vi "Frequency Response - Digital Mic.vi"() -> ()   [LabVIEW 2022 SP3]
uses:
  <vilib>/PDM Acquisition Toolkit/host/Classes/Session/Controls/Logic Levels.ctl
  <vilib>/PDM Acquisition Toolkit/shared/controls/decimation order.ctl
  <vilib>/PDM Acquisition Toolkit/host/Classes/Tasks/PDM Tasks/Controls/Acquisition Mode.ctl
  <vilib>/PDM Acquisition Toolkit/shared/controls/clock mode.ctl
  <vilib>/PDM Acquisition Toolkit/host/API/Controls/PDM Digital Start Trigger Cluster.ctl
  <vilib>/PDM Acquisition Toolkit/shared/controls/PXI trigger lines.ctl
  <vilib>/PDM Acquisition Toolkit/shared/controls/trigger polarity.ctl
  source/shared/measurements/controls/units settings - mic.ctl
  source/shared/measurements/controls/measurement units.ctl
  source/shared/measurements/controls/single tone microphone measurement settings.ctl
  <vilib>/addons/_NISVFA/_Generation/Signal Generation/SV Signal/SV Signal.lvclass/SV Signal.ctl
  <vilib>/DAQmx/write.llb/DAQmx Write (Analog Wfm 1Chan NSamp).vi
  <vilib>/DAQmx/read.llb/DAQmx Read (Analog 1D Wfm NChan NSamp).vi
  <vilib>/addons/_NISVFA/_Generation/Signal Generation/SV Signal/Write Leading Synchronization Pulse Enable.vi
  <vilib>/addons/_NISVFA/_Generation/Signal Generation/SV Signal/Write Synchronization Pulse Duration.vi
  <vilib>/addons/_NISVFA/_Generation/Signal Generation/SV Signal/Read Total Samples.vi
  Program Files/NI/LVAddons/nisvt/1/examples/Sound and Vibration/Audio Measurements/subVIs/sv_Align Waveforms by Leading Sync Pulse.vi
  <vilib>/addons/_NISVFA/_Generation/Signal Generation/SV Signal/Read Synchronization Pulse Waveform.vi
  <vilib>/addons/_NISVFA/_Shared subVIs/Common/svc_Check for Waveform Parameter Continuity (N Ch).vi
  Program Files/NI/LVAddons/nisvt/1/examples/Sound and Vibration/Audio Measurements/subVIs/sv_Append Virtual Reference.vi
  <vilib>/addons/_NISVFA/_Generation/Signal Generation/SV Signal/Calculate Number of Remaining Samples.vi
  Program Files/NI/LVAddons/nisvt/1/examples/Sound and Vibration/Audio Measurements/subVIs/sv_Measure Delay for Active and Idle Channels.vi
  <vilib>/addons/_NISVFA/_Generation/Signal Generation/SV Signal/Read Leading Synchronization Pulse Enable.vi
  <vilib>/addons/_NISVFA/_Generation/Signal Generation/SV Signal/Read Trailing Synchronization Pulse Enable.vi
  <vilib>/addons/_NISVFA/_Shared subVIs/Common/svc_Check for Waveform Parameter Continuity (no state).vi
  <vilib>/addons/_NISVFA/_Shared subVIs/Common/sv_Get NI Property Name String.vi
  <vilib>/addons/Sound and Vibration/svt_Calibration/SV Measure Delay and Polarity and Coherence (Nx1).vi
  Program Files/NI/LVAddons/nisvt/1/examples/Sound and Vibration/Audio Measurements/subVIs/sv_Assign Delay to Idle Channels.vi
  <vilib>/addons/_NISVFA/_Shared subVIs/Common/svc_Get SV Channel Info.vi
  <vilib>/addons/Sound and Vibration/svt_Calibration/SV Measure Delay and Polarity and Coherence.vi
  <vilib>/addons/_NISVFA/_Shared subVIs/Common/svc_Unit Label to Engineering Units.vi
  <vilib>/addons/_NISVFA/_Shared subVIs/Common/svc_Engineering Units to Unit Label.vi
  <vilib>/Analysis/_algsub.llb/Vector Norm.vi
  <vilib>/Analysis/_algsub.llb/Real Vector Norm.vi
  <vilib>/addons/_NISVFA/_Shared subVIs/Common/SV Get Data Subset.vi
  <vilib>/addons/_NISVFA/_Shared subVIs/Common/svc_Get Array Subset (Index).vi
  <vilib>/addons/_NISVFA/_Shared subVIs/Common/svc_Coerce Index and Length.vi
  <vilib>/addons/_NISVFA/_Shared subVIs/Common/svc_Conditional Merge Error.vi
  <vilib>/addons/_NISVFA/_Generation/Signal Generation/SV Discrete Sweep/SV Discrete Sweep.lvclass
  C:/Program Files/NI/LVAddons/nisvt/1/vi.lib/addons/_NISVFA/_Generation/Signal Generation/SV Signal/SV Signal.lvclass
  C:/Program Files/NI/LVAddons/nisvt/1/vi.lib/addons/_NISVFA/_Generation/Signal Generation/SV Function/SV Function.lvclass
  <vilib>/addons/_NISVFA/_Generation/Signal Generation/SV Discrete Sweep/Configure Frequency Sweep at Constant Amplitude.vi
  <vilib>/PDM Acquisition Toolkit/host/API/Public/Create Tasks/Create PDM Input Task.vi
  <vilib>/addons/_NISVFA/_Generation/Signal Generation/SV Signal/Write Ramp Parameters.vi
  <vilib>/addons/_NISVFA/_Generation/Signal Generation/SV Signal/Write Measurement Duration.vi
  <vilib>/addons/_NISVFA/_Generation/Signal Generation/SV Function/Write Measurement Cycles.vi
  <vilib>/addons/_NISVFA/_Generation/Signal Generation/SV Signal/Write Pre-Measurement Settling Duration.vi
  <vilib>/addons/_NISVFA/_Generation/Signal Generation/SV Function/Write Pre-Measurement Settling Cycles.vi
  <vilib>/addons/_NISVFA/_Generation/Signal Generation/SV Signal/Read Sample Rate.vi
  <vilib>/addons/_NISVFA/_Generation/Signal Generation/SV Signal/Read Generation State.vi
  <vilib>/addons/_NISVFA/_Generation/Signal Generation/SV Signal/Read System Timing Model.vi
  <vilib>/PDM Acquisition Toolkit/host/API/Public/Configure/Timing/Configure Timing - PDM Input.vi
  <vilib>/PDM Acquisition Toolkit/host/API/Public/Configure/PDM Channel/Configure Microphone Sensitivity DBFS.vi
  <vilib>/PDM Acquisition Toolkit/host/API/Public/Configure/Triggering/Configure PDM Trigger (Digital Edge).vi
  <vilib>/DAQmx/create/channels.llb/DAQmx Create Channel (AO-Voltage-Basic).vi
  <vilib>/DAQmx/configure/timing.llb/DAQmx Timing (Sample Clock).vi
  <vilib>/DAQmx/configure/events/hardwareSignals.llb/DAQmx Export Signal (Most Signals).vi
  <vilib>/DAQmx/create/channels.llb/DAQmx Create Channel (AI-Sound Pressure-Microphone).vi
  <vilib>/DAQmx/configure/trigger.llb/DAQmx Start Trigger (Digital Edge).vi
  <vilib>/DAQmx/miscellaneous.llb/DAQmx Fill In Error Info.vi
  <vilib>/PDM Acquisition Toolkit/host/API/Public/Read/Read PCM Waveform.vi
  <vilib>/PDM Acquisition Toolkit/host/API/Public/Clear/Clear PDM Input Task.vi
  <vilib>/addons/_NISVFA/_Generation/Signal Generation/SV Signal/Write System Timing Model.vi
  <vilib>/addons/_NISVFA/_Shared subVIs/Data Objects/Waveforms (DBL)/SV Read Newest Data.vi
  <vilib>/measure/maresamp.llb/Resample Waveforms (single shot).vi
  <vilib>/measure/maresamp.llb/Resample Waveform (single shot).vi
  <vilib>/addons/_NISVFA/_Shared subVIs/Common/svc_Check dt for Equal Sample Rates.vi
  <vilib>/Waveform/TSOps.llb/Timestamp Subtract.vi
  <vilib>/Analysis/2dsp.llb/CrossCorrelation.vi
  <vilib>/Analysis/2dsp.llb/1D Cross Correlation (DBL).vi
  <vilib>/addons/_NISVFA/_Shared subVIs/Common/svc_Fit Quadratic to Max Three Points in Array.vi
  <vilib>/Utility/error.llb/Error Cluster From Error Code.vi
  <vilib>/addons/_NISVFA/_Shared subVIs/Common/svc_Caller VI Returned in Error Source.vi
  <vilib>/addons/_NISVFA/_Shared subVIs/Common/SV Remove Delays (1,N) from Waveforms (N Ch) (DBL).vi
  <vilib>/addons/_NISVFA/_Shared subVIs/Common/SV Remove Delays from Waveforms.vi
  <vilib>/addons/_NISVFA/_Shared subVIs/Data Objects/Waveforms (DBL)/SV Read Next Measurement Data.vi
  <vilib>/addons/_NISVFA/_Generation/Signal Generation/SV Signal/SV Signal.lvclass
  <resource>/objmgr/daqmx.rc
  <vilib>/addons/_NISVFA/_Shared subVIs/Data Objects/Waveforms (DBL)/Waveforms (N Ch).lvclass
  Program Files/NI/LVAddons/nisvt/1/examples/Sound and Vibration/SoundVib_Audio Examples.lvlib
  C:/Program Files/NI/LVAddons/nisvt/1/vi.lib/addons/_NISVFA/_Generation/Signal Generation/SV Sinusoid/SV Sinusoid.lvclass
  C:/Program Files/NI/LVAddons/nisvt/1/vi.lib/addons/_NISVFA/_Generation/Signal Generation/SV Discrete Sweep/SV Discrete Sweep.lvclass
  <vilib>/PDM Acquisition Toolkit/host/API/PDM Acquisition Toolkit.lvlib
  <vilib>/PDM Acquisition Toolkit/host/Classes/Tasks/PDM Tasks/PDM Task.lvclass
  <vilib>/PDM Acquisition Toolkit/shared/PDM Shared.lvlib
  <vilib>/PDM Acquisition Toolkit/host/Classes/Session/DecoderSession.lvclass
panel:
  out "duration (s)":dbl
  out "Sample Rate (Hz)":dbl
  in  "Tab Control":T1(tab)=enum."Frequency Response"
  out "Waveform Graph":waveform(dbl)[](graph)=[{"t0"=timestamp(3812131384.799704 s since 1904-01-01), "dt"=1.9531249997269942e-05, "Y"=array[65939 elements], "attributes"=variant("NI_ChannelName"=variant(string "PXI1Slot2/ai0"), "NI_UnitDescription"=variant(string "Pascals"), "NI_dBReference"=variant(dbl 2e-05))}]
  out "XY Graph":cluster{"X":dbl[], "Y":dbl[]}[](graph)
  out "Distortion":cluster{"X":dbl[], "Y":dbl[]}[](graph)
  in  "sweep settings":T2(tab)=enum."Source Settings"
  in  "PDM Channels":string="PXI1Slot5\\PDMi 0"
  in  "Logic Level":T3
  in  "Decimation Factor":T4=64 items=["24"=24, "32"=32, "48"=48, "64"=64, "96"=96, "128"=128]
  in  "PDM Clock Rate":dbl=3072000.0 format="%#_6p"
  in  "Microphone Sensitivity (dBFS)":dbl=-26.0 format="%#_13g"
  out "Actual PDM Clock Rate":dbl=3071999.9922439456 format="%#_6p"
  out "Actual PCM Clock Rate":dbl=47999.99987881165 format="%#_6p"
  in  "physical channels":tag
  in  "microphone sensitivity":dbl=10.0
  in  "number of steps":i32=50 min=1
  in  "amplitude":dbl=94.0 format="%.2p dBSPL"
  in  "frequency spacing":enum16{"Linear", "Logarithmic"}(ring)=enum."Logarithmic"
  in  "sweep range":cluster{"start":dbl, "stop":dbl}={"start"=10000.0, "stop"=300.0} {"stop" min=0.0 format="%.2f"; "start" min=0.0 format="%.2f"}
  in  "output voltage ratio":dbl=0.914 format="%#_g Pa/V"
  in  "speaker excitation channel":tag="PXI1Slot2/ao0"
  in  "measurement":cluster{"time":dbl, "cycles":dbl}={"time"=0.001, "cycles"=25.0} {"cycles" min=5.0 max=1000.0 step=1.0; "time" min=0.0 max=5.0 step=0.0001 format="%.3f s"}
  in  "settling":cluster{"time":dbl, "cycles":dbl}={"time"=0.0, "cycles"=1.0} {"cycles" min=0.0 max=100.0 step=0.5; "time" min=0.0 max=5.0 step=0.0001 format="%.3f s"}
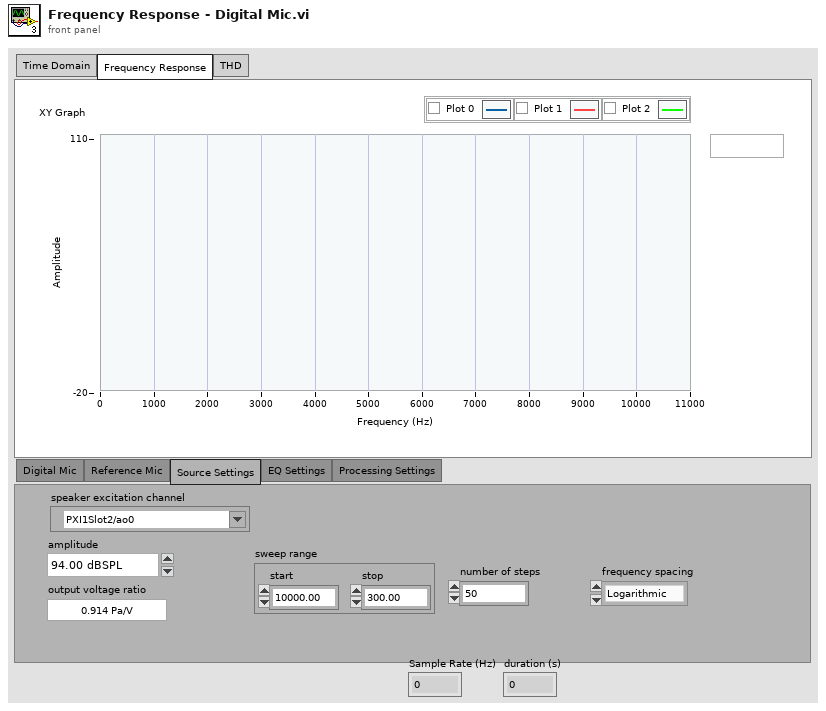
[diagram p1: front panel]
types:
  T1 = enum32{"Time Domain", "Frequency Response", "THD"}
  T2 = enum32{"Digital Mic", "Reference Mic", "Source Settings", "EQ Settings", "Processing Settings"}
  T3 = typedef "PDM Acquisition Class Library.lvlib/DecoderSession.lvclass/Logic Levels.ctl" = enum16{"3.3 V", "1.8 V", "1.2 V"}
  T4 = typedef "PDM Shared.lvlib/decimation order.ctl" = u16
  T5 = typedef "PDM Acquisition Toolkit.lvlib/PDM Digital Start Trigger Cluster.ctl" = cluster{"source":T6, "polarity":T7}
  T6 = typedef "PDM Shared.lvlib/PXI trigger lines.ctl" = enum16{"PXI_Trig0", "PXI_Trig1", "PXI_Trig2", "PXI_Trig3", "PXI_Trig4", "PXI_Trig5", "PXI_Trig6", "PXI_Trig7"}
  T7 = typedef "PDM Shared.lvlib/trigger polarity.ctl" = enum16{"Rising Edge", "Falling Edge"}
  T8 = typedef "PDM Shared.lvlib/clock mode.ctl" = enum16{"divided clock", "DDS"}
  T9 = typedef "PDM Acquisition Class Library.lvlib/PDM Task.lvclass/Acquisition Mode.ctl" = enum16{"Finite", "Continuous"}
  T10 = cluster{"profile":enum16{"Linear", "Half cosine"}, "durations [s]":cluster{"ramp-up":dbl, "transition":dbl, "ramp-down":dbl}}
  T11 = typedef "single tone microphone measurement settings.ctl" = cluster{"Band start":dbl, "Band stop":dbl, "Frequency":dbl}
  T12 = typedef "units settings - mic.ctl" = cluster{"SNR units":T13, "THD+N units":T13, "THD units":T13}
  T13 = typedef "measurement units.ctl" = enum32{"dB", "%", "x/y"}
  T14 = typedef "single tone microphone measurements.ctl" = cluster{"channel":string, "frequency (Hz)":dbl, "amplitude (Pa rms)":dbl, "amplitude (dBSPL)":dbl, "SNR":dbl, "THD+N":dbl, "THD":dbl, "phase (deg)":dbl}
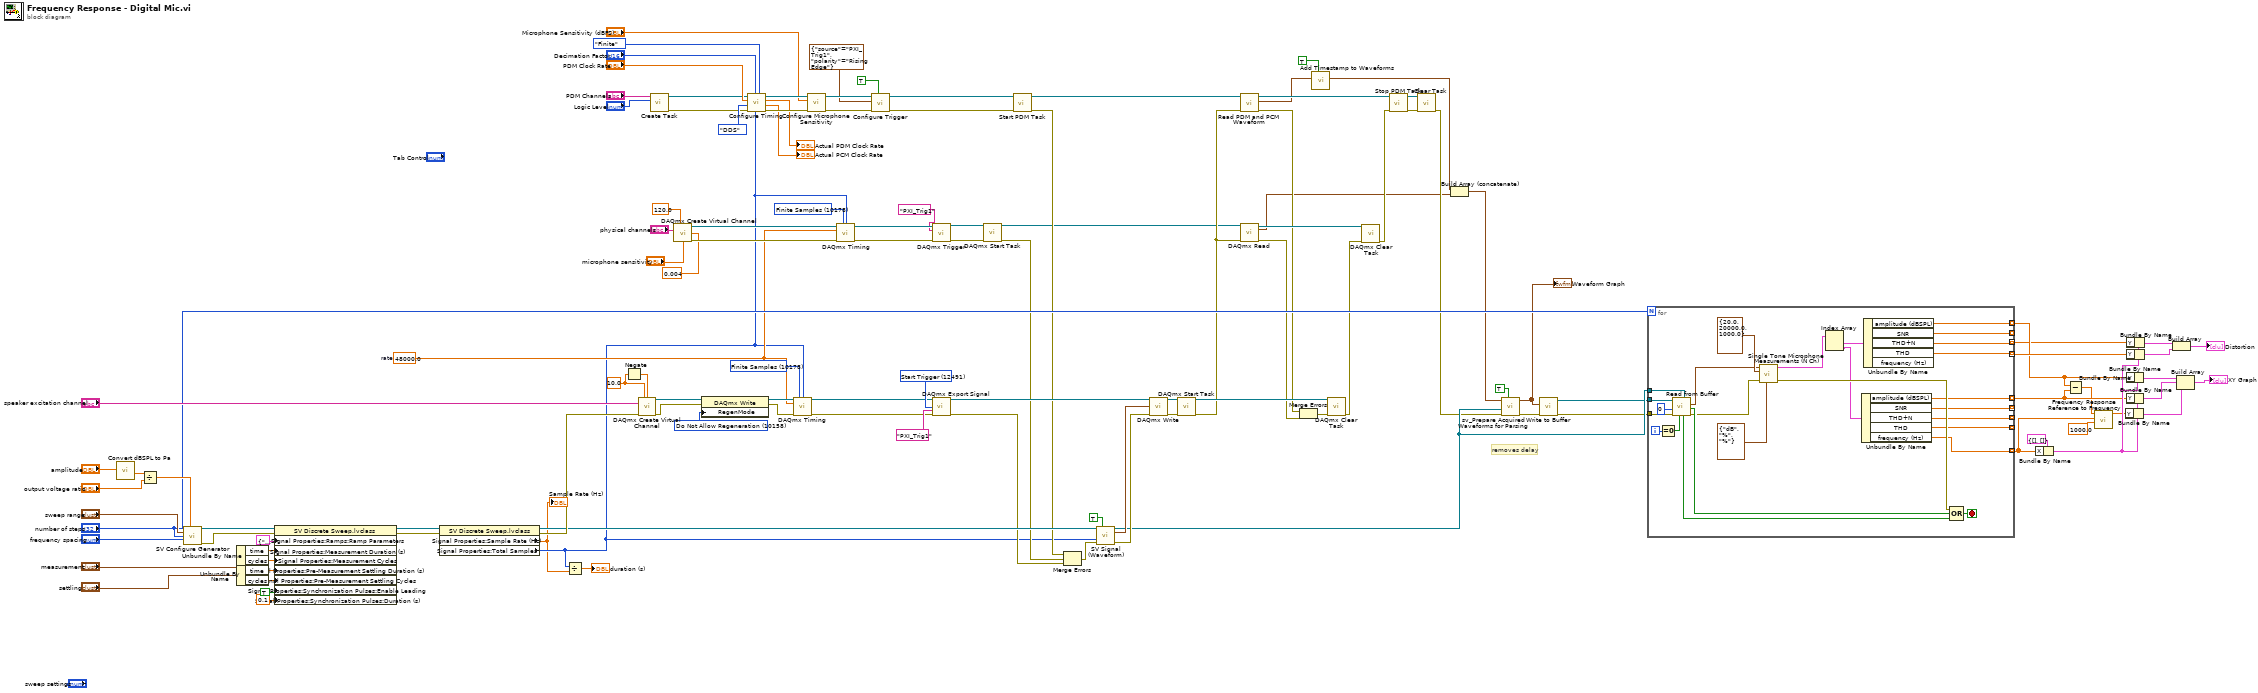
[diagram p0: block diagram]
diagram:
  w44 = 10178 items=["Finite Samples"=10178, "Continuous Samples"=10123, "Hardware Timed Single Point"=12522] ("sample mode")
  w80 = 12491 items=["AI Convert Clock"=12484, "10MHz Reference Clock"=12536, "20MHz Timebase Clock"=12486, "Sample Clock"=12487, "Advance Trigger"=12488, "Reference Trigger"=12490, "Start Trigger"=12491, "Advance Complete Event"=12492, "AI Hold Complete Event"=12493, "Counter Output Event"=12494, "Change Detection Event"=12511, "Watchdog Timer Expired Event"=12512] ("signal")
  w105 = 10158 items=["Allow Regeneration"=10097, "Do Not Allow Regeneration"=10158] ("RegenMode")
  w107 = 10.0 ("maximum value")
  w108 = 10178 items=["Finite Samples"=10178, "Continuous Samples"=10123, "Hardware Timed Single Point"=12522] ("sample mode")
  w39 = 48000.0  # rate
  # "removes delay"
  n1 = call "Convert dBSPL to Pa.vi"("dB SPL"="amplitude") -> ("Pa pk"=w81:dbl)  [unwired: 9 in, 1 out]
  n2 = Divide(x=w81, y="output voltage ratio") -> (x/y=w109:dbl)
  n3 = call-poly <vilib>:"SV Configure Generator.vi"("amplitude"=w109, "frequency range [Hz]"="sweep range", "number of steps"="number of steps", "profile"="frequency spacing") -> ("signal configuration"=w117:refnum<class "SV Discrete Sweep.lvclass">, "error out"=w116:errorcluster)  [unwired: 10 in]
  n4 = Unbundle By Name("measurement") -> ("time"=w119:dbl, "cycles"=w118:dbl)
  n5 = Unbundle By Name("settling") -> ("time"=w121:dbl, "cycles"=w120:dbl)
  n6 = property class="SV Discrete Sweep.lvclass"(reference=w117, error in=w116, "Signal Properties:Ramps:Ramp Parameters"=T10 {"profile"=enum."Half cosine", "durations [s]"={"ramp-up"=0.01, "transition"=0.0, "ramp-down"=0.01}} ("Ramp Parameters"), "Signal Properties:Measurement Duration (s)"=w119, "Signal Properties:Measurement Cycles"=w118, "Signal Properties:Pre-Measurement Settling Duration (s)"=w121, "Signal Properties:Pre-Measurement Settling Cycles"=w120, "Signal Properties:Synchronization Pulses:Enable Leading"=TRUE ("Synchronization Pulses:Enable Leading"), "Signal Properties:Synchronization Pulses:Duration (s)"=0.1 ("Synchronization Pulses:Duration")) -> (reference out=w97:refnum<class "SV Discrete Sweep.lvclass">, error out=w98:errorcluster)
  n7 = property on="Property Node" class="SV Discrete Sweep.lvclass"(reference=w97, error in=w98) -> (reference out=w94:refnum<class "SV Discrete Sweep.lvclass">, error out=w96:errorcluster, "Signal Properties:Sample Rate (Hz)"=w2:dbl, "Signal Properties:Total Samples"=w3:i32)
  "Sample Rate (Hz)" <- w2
  n8 = Divide(x=w3, y=w2) -> (x/y=→"duration (s)":dbl)
  n9 = Negate(x=w107) -> (-x=w106:dbl)
  n10 = call-poly <vilib>:"DAQmx Create Virtual Channel.vi"("maximum value"=w107, "minimum value"=w106, "physical channels"="speaker excitation channel", "error in"=w96) -> ("task out"=w104:refnum<k21>, "error out"=w102:errorcluster)  [unwired: 10 in]
  n11 = call-poly <vilib>:"Create Task.vi"("logic level"="Logic Level", "channel list"="PDM Channels") -> ("error out"=w64:errorcluster, "PDM input task out"=w65:refnum<data-value>)  [unwired: 8 in]
  n12 = call-poly <vilib>:"DAQmx Create Virtual Channel.vi"("maximum sound pressure level"=120.0, "physical channels"="physical channels", "current excitation value"=0.004, "microphone sensitivity"="microphone sensitivity") -> ("task out"=w46:refnum<k21>, "error out"=w45:errorcluster)  [unwired: 10 in]
  n13 = property class="DAQmx Write"(reference=w104, error in=w102, "RegenMode"=w105) -> (reference out=w103:refnum<k21>, error out=w101:errorcluster)
  n14 = call-poly <vilib>:"Configure Timing.vi"("acquisition mode"=Acquisition_Mode."Finite" ("Acquisition Mode"), "number of PCM samples"=w3, "decimation factor"="Decimation Factor", "error in"=w64, "clock mode"=clock_mode."DDS" ("Clock Type"), "PDM clock rate"="PDM Clock Rate", "PDM input task in"=w65) -> ("error out"=w67:errorcluster, "actual PCM clock rate"=→"Actual PCM Clock Rate":dbl, "actual PDM clock rate"=→"Actual PDM Clock Rate":dbl, "PDM input task out"=w68:refnum<data-value>)  [unwired: 1 in]
  n15 = call-poly <vilib>:"DAQmx Timing.vi"("task/channels in"=w103, "sample mode"=w108, "samples per channel"=w3, "rate"=w39, "error in"=w101) -> ("task out"=w76:refnum<k21>, "error out"=w75:errorcluster)  [unwired: 9 in]
  n16 = call-poly <vilib>:"Configure Microphone Sensitivity.vi"("error in"=w67, "microphone sensitivity (dBFS)"="Microphone Sensitivity (dBFS)", "PDM input task in"=w68) -> ("error out"=w58:errorcluster, "PDM input task out"=w61:refnum<data-value>)  [unwired: 7 in]
  n17 = call-poly <vilib>:"DAQmx Timing.vi"("task/channels in"=w46, "sample mode"=w44, "samples per channel"=w3, "rate"=w39, "error in"=w45) -> ("task out"=w38:refnum<k21>, "error out"=w37:errorcluster)  [unwired: 9 in]
  n18 = call-poly <vilib>:"Configure Trigger.vi"("remove filter delay samples"=TRUE, "error in"=w58, "trigger configuration"=T5 {"source"=enum."PXI_Trig1", "polarity"=enum."Rising Edge"}, "PDM input task in"=w61) -> ("error out"=w59:errorcluster, "PDM input task out"=w60:refnum<data-value>)  [unwired: 6 in]
  n19 = call-poly <vilib>:"DAQmx Export Signal.vi"("task/channels in"=w76, "signal"=w80, "output terminal"="PXI_Trig1", "error in"=w75) -> ("task out"=w78:refnum<k21>, "error out"=w77:errorcluster)  [unwired: 10 in]
  n20 = call-poly <vilib>:"DAQmx Trigger.vi"("task/channels in"=w38, "source"="PXI_Trig1", "error in"=w37) -> ("task out"=w34:refnum<k21>, "error out"=w35:errorcluster)  [unwired: 11 in]
  n21 = call <vilib>:"DAQmx Start Task.vi"("task/channels in"=w34, "error in"=w35) -> ("task out"=w30:refnum<k21>, "error out"=w32:errorcluster)  [unwired: 12 in]
  n22 = call <vilib>:"Start PDM Task.vi"("error in"=w59, "PDM input task in"=w60) -> ("error out"=w33:errorcluster, "PDM input task out"=w72:refnum<data-value>)  [unwired: 8 in]
  n23 = Merge Errors(w33, w32, w77) -> (w93:errorcluster)
  n24 = call-dynamic "SV Signal (Waveform).vi"("signal configuration"=w94, "reset"=TRUE, "samples"=w3, "error in (no error)"=w93) -> ("signal configuration"=w85:refnum<class "SV Discrete Sweep.lvclass">, "output waveform"=w91:waveform(dbl), "error out"=w92:errorcluster)  [unwired: 6 in, 3 out]
  n25 = call-poly <vilib>:"DAQmx Write.vi"("task/channels in"=w78, "data"=w91, "error in"=w92) -> ("task out"=w89:refnum<k21>, "error out"=w90:errorcluster)  [unwired: 10 in, 1 out]
  n26 = call <vilib>:"DAQmx Start Task.vi"("task/channels in"=w89, "error in"=w90) -> ("task out"=w88:refnum<k21>, "error out"=w31:errorcluster)  [unwired: 12 in]
  n27 = call-poly <vilib>:"Read PDM and PCM Waveform.vi"("error in"=w31, "PDM input task in"=w72) -> ("error out"=w25:errorcluster, "PCM waveforms"=w48:waveform(dbl)[], "PDM input task out"=w51:refnum<data-value>)  [unwired: 6 in, 1 out]
  n28 = call-poly <vilib>:"DAQmx Read.vi"("task/channels in"=w30, "error in"=w31) -> ("task out"=w28:refnum<k21>, "data"=w23:waveform(dbl)[], "error out"=w24:errorcluster)  [unwired: 11 in]
  n29 = Merge Errors(w25, w24) -> (w26:errorcluster)
  n30 = call "Add Timestamp to Waveforms.vi"("initialize"=TRUE, "waveforms"=w48) -> ("waveforms"=w21:waveform(dbl)[])  [unwired: 9 in]
  n31 = call <vilib>:"DAQmx Clear Task.vi"("task in"=w88, "error in"=w26) -> ("error out"=w27:errorcluster)  [unwired: 13 in]
  n32 = call <vilib>:"DAQmx Clear Task.vi"("task in"=w28, "error in"=w27) -> ("error out"=w29:errorcluster)  [unwired: 13 in]
  n33 = call <vilib>:"Stop PDM Task.vi"("error in"=w29, "PDM input task in"=w51) -> ("error out"=w53:errorcluster, "PDM input task out"=w54:refnum<data-value>)  [unwired: 8 in]
  n34 = call-poly <vilib>:"Clear Task.vi"("error in"=w53, "PDM input task in"=w54) -> ("error out"=w52:errorcluster)  [unwired: 9 in]
  n35 = Build Array (concatenate)(w21, w23) -> (w20:waveform(dbl)[])
  n36 = call "sv_Prepare Acquired Waveforms for Parsing.vi"("restart (F)"=TRUE, "error in"=w52, "SV Signal"=w85, "acquired channel waveforms"=w20) -> ("error out"=w86:errorcluster, "aligned channel waveforms"=w22:waveform(dbl)[])  [unwired: 5 in, 1 out]
  "Waveform Graph" <- w22
  n37 = call <vilib>:"Write to Buffer.vi"("error in (no error)"=w86, "waveforms"=w22) -> ("error out"=w50:errorcluster, "buffer out"=w84:refnum<data-value>)  [unwired: 7 in, 1 out]
  n38 = for {
    N: "number of steps" -> [_]
    tunnel: w84 -> [w146]
    tunnel: w85 -> [w145]
    tunnel: w50 -> [w144]
    tunnel: [w126] -> w8 mode=indexing
    tunnel: [w127] -> w7 mode=indexing
    tunnel: [w135] -> w6 mode=indexing
    tunnel: [w134] -> _ mode=indexing
    tunnel: [w133] -> w4 mode=indexing
    tunnel: [w132] -> w16 mode=indexing
    tunnel: [w125] -> _ mode=indexing
    tunnel: [w124] -> _ mode=indexing
    tunnel: [w123] -> _ mode=indexing
    i -> [w141]
    stop <- w142 stop-if-true
    n39 = Equal To 0?(x=w141) -> (x = 0?=w140:bool)
    n40 = call-poly <vilib>:"Read from Buffer.vi"("test signal configuration"=w145, "reset start (F)"=w140, "error in (no error)"=w144, "timeout (1000 ms)"=0, "buffer"=w146) -> ("error out"=w139:errorcluster, "end of buffer"=w143:bool, "waveforms subset"=w129:waveform(dbl)[], "done"=w148:bool)  [unwired: 2 in, 1 out]
    n41 = call "Single Tone Microphone Measurements (N Ch).vi"("units settings"=T12 {"SNR units"=enum."dB", "THD+N units"=enum."%", "THD units"=enum."%"}, "error in"=w139, "measurement settings"=T11 {"Band start"=20.0, "Band stop"=20000.0, "Frequency"=1000.0}, "waveforms"=w129) -> ("error out"=w138:errorcluster, "measurements"=w137:T14[])  [unwired: 4 in, 2 out]
    n42 = Index Array(array=w137) -> (element #1=w136:T14, element #2=w128:T14)  [unwired: 2 in]
    n43 = Unbundle By Name(w128) -> ("amplitude (dBSPL)"=w127:dbl, "SNR"=w123:dbl, "THD+N"=w124:dbl, "THD"=w125:dbl, "frequency (Hz)"=w126:dbl)
    n44 = Unbundle By Name(w136) -> ("amplitude (dBSPL)"=w135:dbl, "SNR"=w134:dbl, "THD+N"=w133:dbl, "THD"=w132:dbl)  [unwired: 1 out]
    n45 = Compound Arithmetic op=OR(w138, w143, w148) -> (w142:bool)
  }
  n46 = Bundle By Name(cluster=cluster{"X":dbl[], "Y":dbl[]} {"X"=[], "Y"=[]} ("THD vs Amplitude"), "X"=w8) -> (w10:cluster{"X":dbl[], "Y":dbl[]})
  n47 = Subtract(x=w6, y=w7) -> (x-y=w5:dbl[])
  n48 = call "Frequency Response Reference to Frequency.vi"("reference frequency"=1000.0, "frequency"=w8, "amplitude (dBPL)"=w5) -> ("amplitude (dBr)"=w9:dbl[])  [unwired: 8 in]
  n49 = Bundle By Name(cluster=w10, "Y"=w9) -> (w11:cluster{"X":dbl[], "Y":dbl[]})
  n50 = Bundle By Name(cluster=w10, "Y"=w6) -> (w17:cluster{"X":dbl[], "Y":dbl[]})
  n51 = Bundle By Name(cluster=w10, "Y"=w7) -> (w19:cluster{"X":dbl[], "Y":dbl[]})
  n52 = Bundle By Name(cluster=w10, "Y"=w4) -> (w15:cluster{"X":dbl[], "Y":dbl[]})
  n53 = Bundle By Name(cluster=w10, "Y"=w16) -> (w14:cluster{"X":dbl[], "Y":dbl[]})
  n54 = Build Array(w15, w14) -> (→"Distortion":cluster{"X":dbl[], "Y":dbl[]}[])
  n55 = Build Array(w17, w19, w11) -> (→"XY Graph":cluster{"X":dbl[], "Y":dbl[]}[])
